vi "catalog.wait_until_ingest_complete.vi"(6 "timeout (-1: never)":i32=-1, 8 "error in":errorcluster, 10 "datasetRid":string, 11 "Nominal Client":refnum<class "Nominal Client.lvclass">) -> (0 "error out":errorcluster, 3 "Nominal Client out":refnum<class "Nominal Client.lvclass">)   [LabVIEW 2020, in "Nominal Client.lvclass"]
doc: "Just for datasets"
uses:
  Nominal Client.lvclass
  catalog.get_ingest_progress_v2.vi
  catalog.get_ingest_progress_v2.vi/dd643593-8eee-4817-a06c-cfd53975b380.vi
  <vilib>/Utility/error.llb/Clear Errors.vi
  iso8601_string_to_timestamp.vi
  http.get.vi
  <vilib>/JDP Science/JSONtext/JSON text to Variant.vi
  <vilib>/LabVIEW Open Source Project/Epoch Date & Time/formatter.iso8601/ISO8601 DateString to Timestamp.vi
  <vilib>/JDP Science/JSONtext/LVClass Serializer/JSONtext LVClass Serializer.lvclass
  Nominal Client.lvclass/Nominal Client.ctl
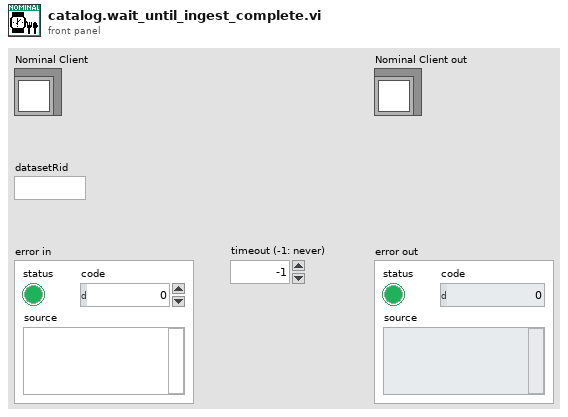
[diagram p1: front panel]
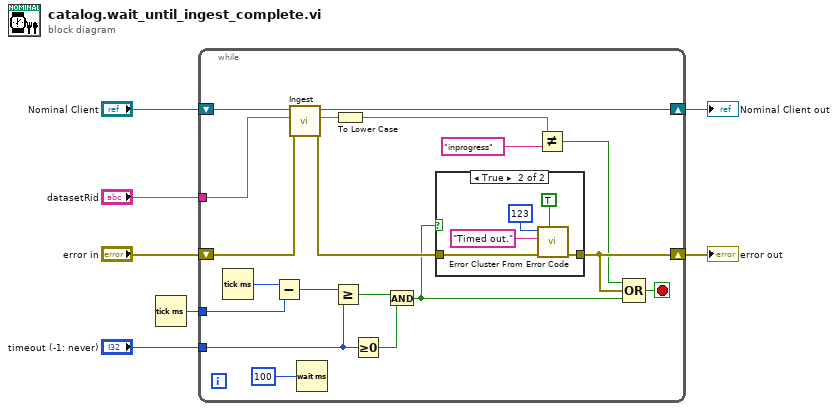
[diagram p0: block diagram]
diagram:
  n1 = Tick Count (ms)() -> (millisecond timer value=w3:u32)
  n2 = while {
    shift-right: [w24] -> w6
    shift-left: "Nominal Client" -> [w26]
    shift-right: [w12] -> w5
    shift-left: "error in" -> [w25]
    tunnel: w3 -> [w20]
    tunnel: "timeout (-1: never)" -> [w18]
    tunnel: "datasetRid" -> [w8]
    stop <- w23 stop-if-true
    n3 = Tick Count (ms)() -> (millisecond timer value=w21:u32)
    n4 = Subtract(x=w21, y=w20) -> (x-y=w19:u32)
    n5 = call-poly "Ingest.vi"("error in"=w25, "datasetRid[]"=w8, "Nominal Client in"=w26) -> ("error out"=w11:errorcluster, "Status"=w15:string, "Nominal Client out"=w24:refnum<class "Nominal Client.lvclass">)  [unwired: 5 in, 1 out]
    n6 = Wait (ms)(milliseconds to wait=u32 100) -> ()  [unwired: 1 out]
    n7 = Greater Or Equal?(x=w19, y=w18) -> (x >= y?=w16:bool)
    n8 = To Lower Case(string=w15) -> (all lower case string=w14:string)
    n9 = Greater Or Equal To 0?(x=w18) -> (x >= 0?=w17:bool)
    n10 = And(x=w16, y=w17) -> (x .and. y?=w10:bool)
    n11 = case shown="True" w10 {
      tunnel: [w27 w29] -> w12
      tunnel: w11 -> [w27 w28]
      frame False {
      }
      frame True {
        n12 = call <vilib>:"Error Cluster From Error Code.vi"("show call chain? (False)"=TRUE, "error in (no error)"=w28, "error message (\"\")"="Timed out." ("error message (\"\")"), "error code (0)"=123) -> ("error out"=w29:errorcluster)  [unwired: 5 in]
      }
    }
    n13 = Not Equal?(x=w14, y="inprogress") -> (x != y?=w9:bool)
    n14 = Compound Arithmetic op=OR(w9, w12, w10) -> (w23:bool)
  }
  "Nominal Client out" <- w6
  "error out" <- w5
